vi "VIH HelpGen - Build Log Handler - Save Log File.vi"(6 "CHM status":T1, 7 "preparation error":errorcluster, 8 "error in":errorcluster, 9 "Menu Help status":T3, 10 "VI Help status":T4, 11 "Status":T2) -> (0 "error out":errorcluster)   [LabVIEW 2014]
doc: "::: VI Helpeks :::\nCopyright (c) 2000-2026 Konstantin Shifershteyn. All rights reserved."
uses:
  <vilib>/Utility/error.llb/DialogType.ctl
panel:
  # "VI Helpeks\nCopyright (c) 2012-2026 Konstantin Shifershteyn"
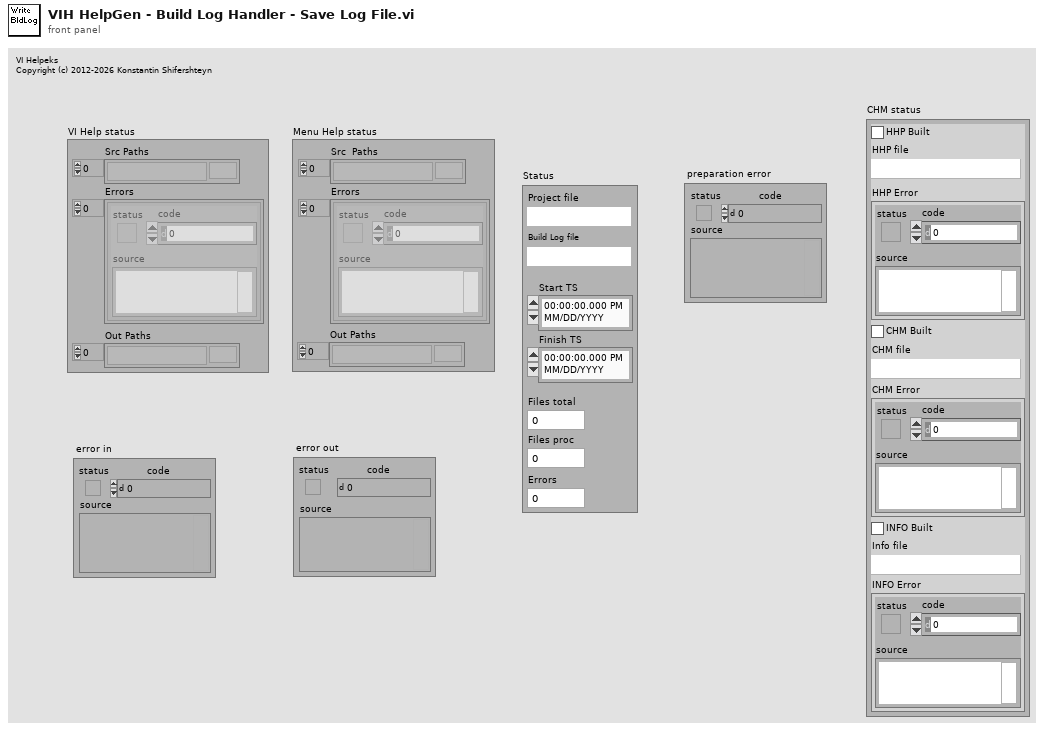
[diagram p1: front panel]
types:
  T1 = cluster{"HHP Built":bool, "HHP file":path, "HHP Error":errorcluster, "CHM Built":bool, "CHM file":path, "CHM Error":errorcluster, "INFO Built":bool, "Info file":path, "INFO Error":errorcluster}
  T2 = cluster{"Project file":path, "Build Log file":path, "Start TS":timestamp, "Finish TS":timestamp, "Files total":i32, "Files proc":i32, "Errors":i32}
  T3 = cluster{"Src  Paths":path[], "Errors":errorcluster[], "Out Paths":path[]}
  T4 = cluster{"Src Paths":path[], "Errors":errorcluster[], "Out Paths":path[]}
  T5 = enum16{"none", "LV description", "VH minimum", "VH extended"}
  T6 = typedef "DialogType.ctl" = u16
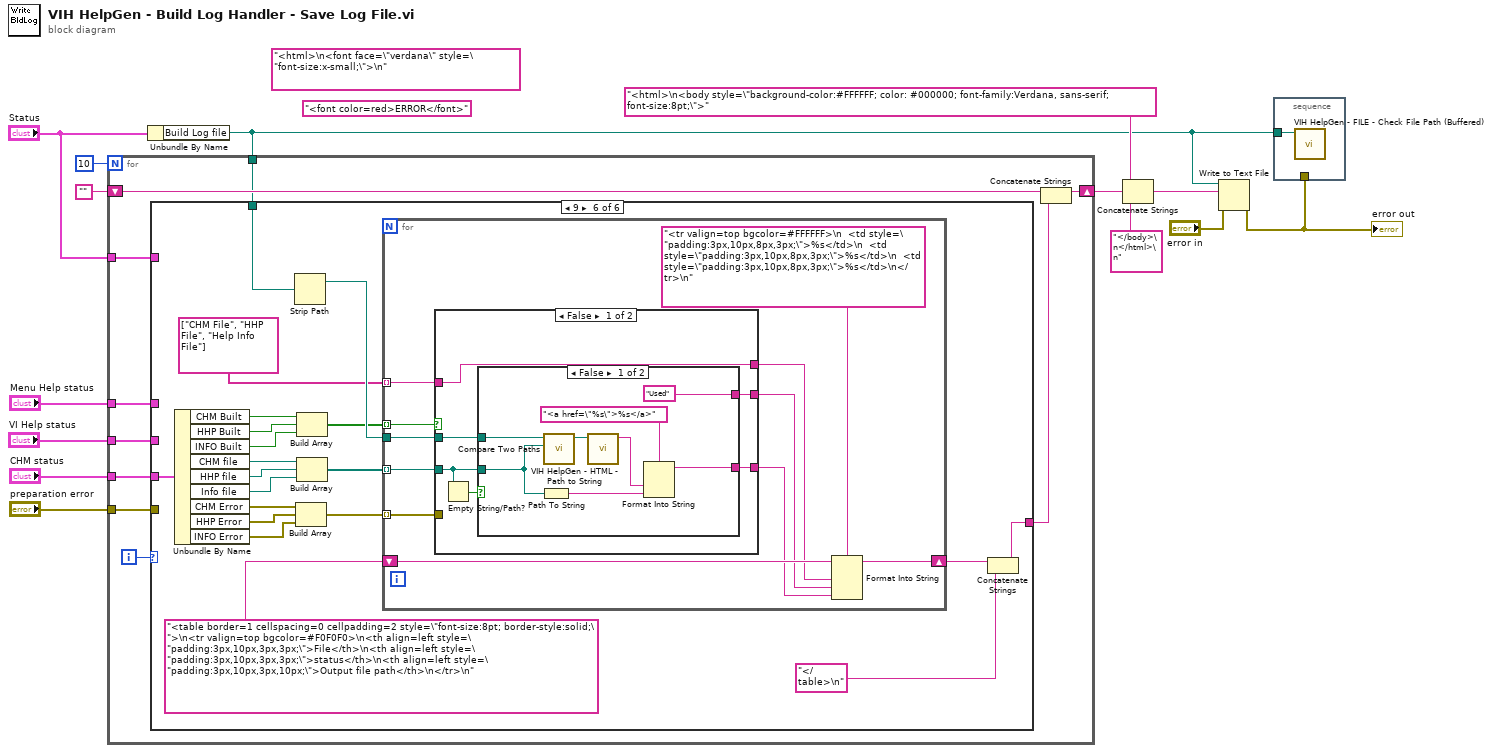
[diagram p0: block diagram]
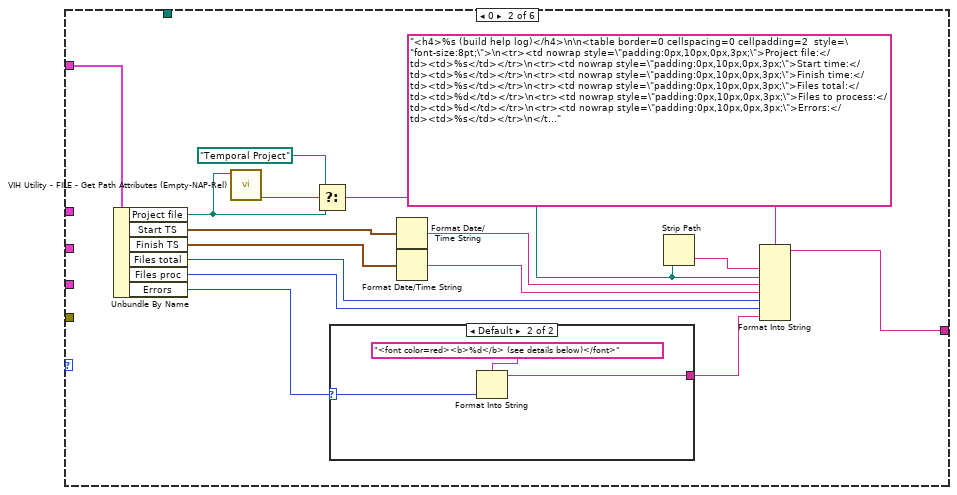
[diagram p3: hidden frame]
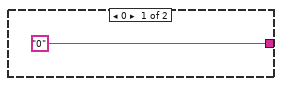
[diagram p4: hidden frame]
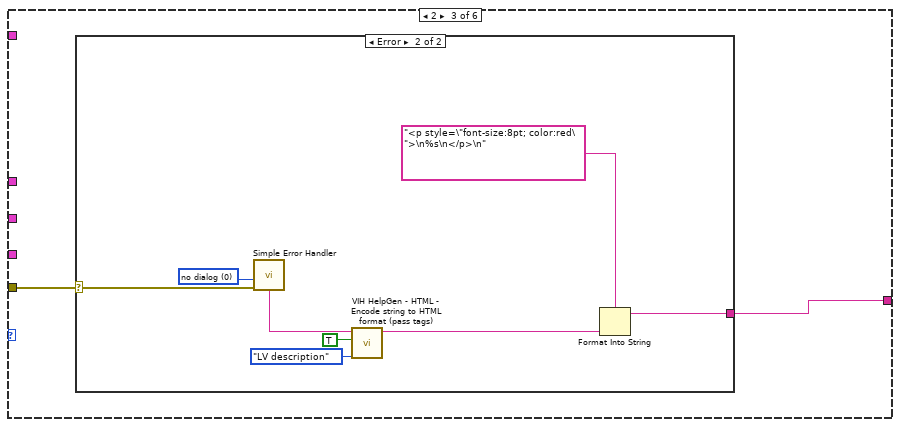
[diagram p5: hidden frame]
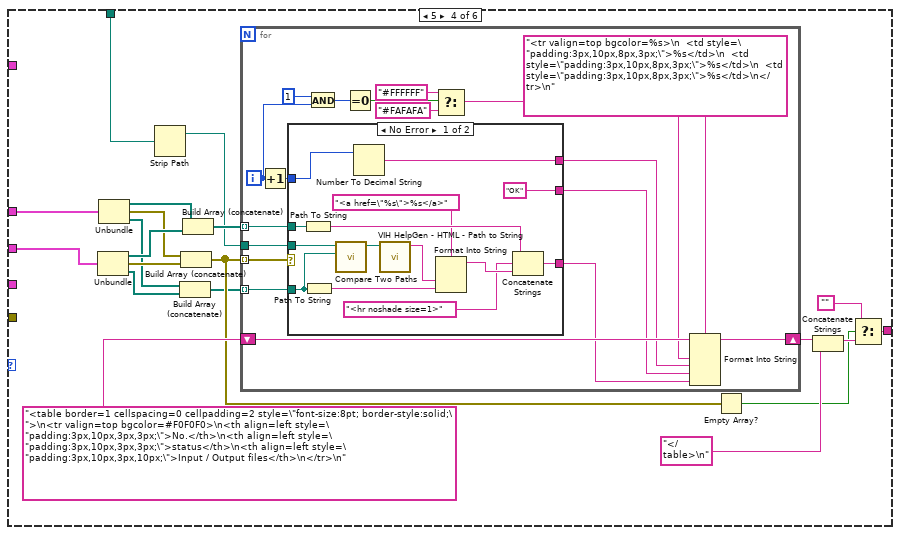
[diagram p7: hidden frame]
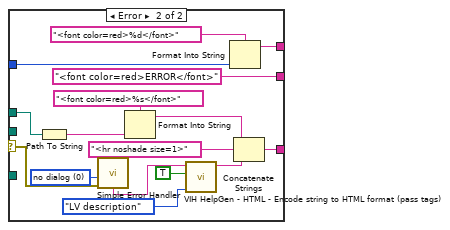
[diagram p8: hidden frame]
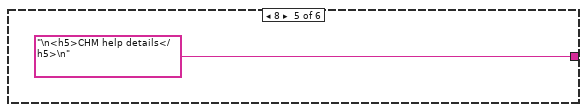
[diagram p9: hidden frame]
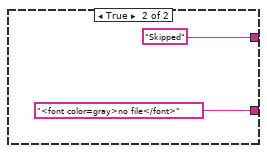
[diagram p10: hidden frame]
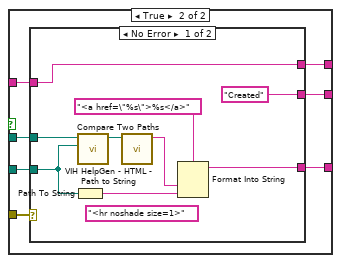
[diagram p11: hidden frame]
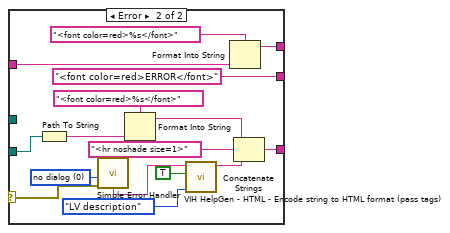
[diagram p12: hidden frame]
diagram:
  (unwired) "<font color=red>ERROR</font>"
  (unwired) "<html>\n<font face=\"verdana\" style=\"font-size:x-small;\">\n"
  n1 = Unbundle By Name("Status") -> ("Build Log file"=w4:path)
  n2 = for {
    N: 10 -> [_]
    shift-right: [w21] -> w14
    shift-left: "" -> [w23]
    tunnel: "Status" -> [w20]
    tunnel: "preparation error" -> [w19]
    tunnel: w4 -> [w18]
    tunnel: "CHM status" -> [w17]
    tunnel: "Menu Help status" -> [w16]
    tunnel: "VI Help status" -> [w15]
    i -> [w24]
    n3 = case shown="9" w24 {
      tunnel: [_ w39 w45 w65 "\n<h5>CHM help details</h5>\n" w131] -> w22
      tunnel: w20 -> [_ w32 _ _ _ _]
      tunnel: w19 -> [_ _ w46 _ _ _]
      tunnel: w18 -> [_ _ _ w58 _ w140]
      tunnel: w17 -> [_ _ _ _ _ w138]
      tunnel: w16 -> [_ _ _ w56 _ _]
      tunnel: w15 -> [_ _ _ w55 _ _]
      frame Default {
      }
      frame 0 {
        n4 = Unbundle By Name(w32) -> ("Project file"=w27:path, "Start TS"=w38:timestamp, "Finish TS"=w36:timestamp, "Files total"=w34:i32, "Files proc"=w33:i32, "Errors"=w30:i32)
        n5 = call "VIH Utility - FILE - Get Path Attributes (Empty-NAP-Rel).vi"("Path"=w27) -> ("Not A Path or Empty path"=w28:bool)  [unwired: 6 in, 4 out]
        n6 = Select(t=path "Temporal Project", s=w28, f=w27) -> (s? t:f=w25:path)
        n7 = case shown="Default" w30 {
          selector: w30 -> [_ w44]
          tunnel: ["0" w43] -> w29
          frame 0 {
          }
          frame Default {
            n8 = Format Into String(format string="<font color=red><b>%d</b> (see details below)</font>", w44) -> (resulting string=w43:string)  [unwired: 2 in, 1 out]
          }
        }
        n9 = Format Date/Time String(seconds (now)=w38) -> (date/time string=w37:string)  [unwired: 2 in]
        n10 = Format Date/Time String(seconds (now)=w36) -> (date/time string=w35:string)  [unwired: 2 in]
        n11 = Strip Path(path=w25) -> (name=w31:string)  [unwired: 1 out]
        n12 = Format Into String(format string="<h4>%s (build help log)</h4>\n\n<table border=0 cellspacing=0 cellpadding=2  style=\"font-size:8pt;\">\n<tr><td nowrap style=\"padding:0px,10px,0px,3px;\">Project file:</td><td>%s</td></tr>\n<tr><td nowrap style=\"padding:0px,10px,0px,3px;\">Start time:</td><td>%s</td></tr>\n<tr><td nowrap style=\"padding:0px,10px,0px,3px;\">Finish time:</td><td>%s</td></tr>\n<tr><td nowrap style=\"padding:0px,10px,0px,3px;\">Files total:</td><td>%d</td></tr>\n<tr><td nowrap style=\"padding:0px,10px,0px,3px;\">Files to process:</td><td>%d</td></tr>\n<tr><td nowrap style=\"padding:0px,10px,0px,3px;\">Errors:</td><td>%s</td></tr>\n</table>\n\n<h5>Build help details:</h5>\n", w31, w25, w37, w35, w34, w33, w29) -> (resulting string=w39:string)  [unwired: 2 in, 1 out]
      }
      frame 2 {
        n13 = case shown="Error" w46 {
          selector: w46 -> [_ w52]
          tunnel: [_ w49] -> w45
          frame No Error {
          }
          frame Error {
            w54 = T6 0 items=["no dialog", "OK message", "continue or stop message", "OK message + warnings", "continue/stop + warnings"] ("type of dialog (OK msg:1)")
            n14 = call <vilib>:"Simple Error Handler.vi"("type of dialog (OK msg:1)"=w54, "error in (no error)"=w52) -> ("message"=w53:string)  [unwired: 3 in, 4 out]
            n15 = call "VIH HelpGen - HTML - Encode string to HTML format (pass tags).vi"("HTML Tagset allowed"=T5."LV description" ("Tag set"), "Reject CR (F)"=TRUE, "string"=w53) -> ("HTML string"=w51:string)  [unwired: 8 in]
            n16 = Format Into String(format string="<p style=\"font-size:8pt; color:red\">\n%s\n</p>\n", w51) -> (resulting string=w49:string)  [unwired: 2 in, 1 out]
          }
        }
      }
      frame 5 {
        n17 = Unbundle(w55) -> ("Src Paths"=w70:path[], "Errors"=w68:errorcluster[], "Out Paths"=w60:path[])
        n18 = Unbundle(w56) -> ("Src  Paths"=w71:path[], "Errors"=w69:errorcluster[], "Out Paths"=w61:path[])
        n19 = Strip Path(path=w58) -> (stripped path=w57:path)  [unwired: 1 out]
        n20 = Build Array (concatenate)(w61, w60) -> (w59:path[])
        n21 = Build Array (concatenate)(w69, w68) -> (w63:errorcluster[])
        n22 = Build Array (concatenate)(w71, w70) -> (w67:path[])
        n23 = for {
          tunnel: w67 -> [w87] mode=indexing
          tunnel: w63 -> [w89] mode=indexing
          shift-right: [w90] -> w74
          shift-left: "<table border=1 cellspacing=0 cellpadding=2 style=\"font-size:8pt; border-style:solid;\">\n<tr valign=top bgcolor=#F0F0F0>\n<th align=left style=\"padding:3px,10px,3px,3px;\">No.</th>\n<th align=left style=\"padding:3px,10px,3px,3px;\">status</th>\n<th align=left style=\"padding:3px,10px,3px,10px;\">Input / Output files</th>\n</tr>\n" -> [w91]
          tunnel: w59 -> [w83] mode=indexing
          tunnel: w57 -> [w82]
          i -> [w81]
          n24 = Increment(x=w81) -> (x+1=w84:i32)
          n25 = case shown="No Error" w89 {
            selector: w89 -> [_ w118]
            tunnel: ["OK" ("f") "<font color=red>ERROR</font>"] -> w88
            tunnel: w87 -> [w105 w121]
            tunnel: [w99 w114] -> w86
            tunnel: [w103 w110] -> w85
            tunnel: w84 -> [w104 w109]
            tunnel: w83 -> [w96 _]
            tunnel: w82 -> [w95 _]
            frame No Error {
              n26 = Path To String(path=w105) -> (string=w98:string)
              n27 = Path To String(path=w96) -> (string=w102:string)
              n28 = call <vilib>:"Compare Two Paths.vi"("Path 2"=w96, "Path 1"=w95) -> ("Relative Path from 1 to 2"=w94:path)  [unwired: 6 in, 3 out]
              n29 = Number To Decimal String(number=w104) -> (decimal integer string=w103:string)  [unwired: 1 in]
              n30 = call "VIH HelpGen - HTML - Path to String.vi"("Path"=w94) -> ("String"=w93:string)  [unwired: 10 in]
              n31 = Format Into String(format string="<a href=\"%s\">%s</a>", w93, w102) -> (resulting string=w101:string)  [unwired: 2 in, 1 out]
              n32 = Concatenate Strings(w98, "<hr noshade size=1>" ("string"), w101) -> (w99:string)
            }
            frame Error {
              w117 = T6 0 items=["no dialog", "OK message", "continue or stop message", "OK message + warnings", "continue/stop + warnings"] ("type of dialog (OK msg:1)")
              n33 = Path To String(path=w121) -> (string=w120:string)
              n34 = call <vilib>:"Simple Error Handler.vi"("type of dialog (OK msg:1)"=w117, "error in (no error)"=w118) -> ("message"=w113:string)  [unwired: 3 in, 4 out]
              n35 = Format Into String(format string="<font color=red>%s</font>", w120) -> (resulting string=w116:string)  [unwired: 2 in, 1 out]
              n36 = call "VIH HelpGen - HTML - Encode string to HTML format (pass tags).vi"("HTML Tagset allowed"=T5."LV description" ("Tag set"), "Reject CR (F)"=TRUE, "string"=w113) -> ("HTML string"=w112:string)  [unwired: 8 in]
              n37 = Format Into String(format string="<font color=red>%d</font>", w109) -> (resulting string=w110:string)  [unwired: 2 in, 1 out]
              n38 = Concatenate Strings(w116, "<hr noshade size=1>" ("string"), w112) -> (w114:string)
            }
          }
          n39 = And(x=1, y=w81) -> (x .and. y?=w79:i32)
          n40 = Equal To 0?(x=w79) -> (x = 0?=w78:bool)
          n41 = Select(t="#FFFFFF", s=w78, f="#FAFAFA") -> (s? t:f=w75:string)
          n42 = Format Into String(format string="<tr valign=top bgcolor=%s>\n  <td style=\"padding:3px,10px,8px,3px;\">%s</td>\n  <td style=\"padding:3px,10px,8px,3px;\">%s</td>\n  <td style=\"padding:3px,10px,8px,3px;\">%s</td>\n</tr>\n", initial string=w91, w75, w85, w88, w86) -> (resulting string=w90:string)  [unwired: 1 in, 1 out]
        }
        n43 = Empty Array?(array=w63) -> (empty?=w62:bool)
        n44 = Concatenate Strings(w74, "</table>\n") -> (w66:string)
        n45 = Select(t="", s=w62, f=w66) -> (s? t:f=w65:string)
      }
      frame 8 {
      }
      frame 9 {
        n46 = Unbundle By Name(w138) -> ("CHM Built"=w129:bool, "HHP Built"=w137:bool, "INFO Built"=w124:bool, "CHM file"=w128:path, "HHP file"=w136:path, "Info file"=w135:path, "CHM Error"=w127:errorcluster, "HHP Error"=w134:errorcluster, "INFO Error"=w125:errorcluster)
        n47 = Strip Path(path=w140) -> (stripped path=w139:path)  [unwired: 1 out]
        n48 = Build Array(w127, w134, w125) -> (w133:errorcluster[])
        n49 = Build Array(w129, w137, w124) -> (w130:bool[])
        n50 = Build Array(w128, w136, w135) -> (w132:path[])
        n51 = for {
          tunnel: w132 -> [w149] mode=indexing
          tunnel: w133 -> [w151] mode=indexing
          shift-right: [w152] -> w143
          shift-left: "<table border=1 cellspacing=0 cellpadding=2 style=\"font-size:8pt; border-style:solid;\">\n<tr valign=top bgcolor=#F0F0F0>\n<th align=left style=\"padding:3px,10px,3px,3px;\">File</th>\n<th align=left style=\"padding:3px,10px,3px,3px;\">status</th>\n<th align=left style=\"padding:3px,10px,3px,10px;\">Output file path</th>\n</tr>\n" -> [w153]
          tunnel: w139 -> [w146]
          tunnel: w130 -> [w145] mode=indexing
          tunnel: string[] ["CHM File", "HHP File", "Help Info File"] -> [w144] mode=indexing
          n52 = case shown="False" w145 {
            tunnel: w151 -> [_ w177]
            tunnel: [w159 w176] -> w150
            tunnel: w149 -> [w155 w175]
            tunnel: [w158 w174] -> w148
            tunnel: [w160 w173] -> w147
            tunnel: w144 -> [w160 w172]
            tunnel: w146 -> [w156 w171]
            frame False {
              n53 = Empty String/Path?(string/path=w155) -> (empty?=w157:bool)
              n54 = case shown="False" w157 {
                tunnel: ["Used" "Skipped"] -> w159
                tunnel: [w161 "<font color=gray>no file</font>"] -> w158
                tunnel: w156 -> [w163 _]
                tunnel: w155 -> [w162 _]
                frame False {
                  n55 = Path To String(path=w162) -> (string=w167:string)
                  n56 = call <vilib>:"Compare Two Paths.vi"("Path 2"=w162, "Path 1"=w163) -> ("Relative Path from 1 to 2"=w165:path)  [unwired: 6 in, 3 out]
                  n57 = call "VIH HelpGen - HTML - Path to String.vi"("Path"=w165) -> ("String"=w164:string)  [unwired: 10 in]
                  n58 = Format Into String(format string="<a href=\"%s\">%s</a>", w164, w167) -> (resulting string=w161:string)  [unwired: 2 in, 1 out]
                }
                frame True {
                }
              }
            }
            frame True {
              n59 = case shown="No Error" w177 {
                selector: w177 -> [_ w198]
                tunnel: ["Created" ("f") "<font color=red>ERROR</font>"] -> w176
                tunnel: w175 -> [w180 w201]
                tunnel: [w178 w194] -> w174
                tunnel: [w179 w190] -> w173
                tunnel: w172 -> [w179 w189]
                tunnel: w171 -> [w183 _]
                frame No Error {
                  (unwired) "<hr noshade size=1>" ("string")
                  n60 = Path To String(path=w180) -> (string=w185:string)
                  n61 = call <vilib>:"Compare Two Paths.vi"("Path 2"=w180, "Path 1"=w183) -> ("Relative Path from 1 to 2"=w182:path)  [unwired: 6 in, 3 out]
                  n62 = call "VIH HelpGen - HTML - Path to String.vi"("Path"=w182) -> ("String"=w181:string)  [unwired: 10 in]
                  n63 = Format Into String(format string="<a href=\"%s\">%s</a>", w181, w185) -> (resulting string=w178:string)  [unwired: 2 in, 1 out]
                }
                frame Error {
                  w197 = T6 0 items=["no dialog", "OK message", "continue or stop message", "OK message + warnings", "continue/stop + warnings"] ("type of dialog (OK msg:1)")
                  n64 = Path To String(path=w201) -> (string=w200:string)
                  n65 = call <vilib>:"Simple Error Handler.vi"("type of dialog (OK msg:1)"=w197, "error in (no error)"=w198) -> ("message"=w193:string)  [unwired: 3 in, 4 out]
                  n66 = Format Into String(format string="<font color=red>%s</font>", w200) -> (resulting string=w196:string)  [unwired: 2 in, 1 out]
                  n67 = call "VIH HelpGen - HTML - Encode string to HTML format (pass tags).vi"("HTML Tagset allowed"=T5."LV description" ("Tag set"), "Reject CR (F)"=TRUE, "string"=w193) -> ("HTML string"=w192:string)  [unwired: 8 in]
                  n68 = Format Into String(format string="<font color=red>%s</font>", w189) -> (resulting string=w190:string)  [unwired: 2 in, 1 out]
                  n69 = Concatenate Strings(w196, "<hr noshade size=1>" ("string"), w192) -> (w194:string)
                }
              }
            }
          }
          n70 = Format Into String(format string="<tr valign=top bgcolor=#FFFFFF>\n  <td style=\"padding:3px,10px,8px,3px;\">%s</td>\n  <td style=\"padding:3px,10px,8px,3px;\">%s</td>\n  <td style=\"padding:3px,10px,8px,3px;\">%s</td>\n</tr>\n", initial string=w153, w147, w150, w148) -> (resulting string=w152:string)  [unwired: 1 in, 1 out]
        }
        n71 = Concatenate Strings(w143, "</table>\n") -> (w131:string)
      }
    }
    n72 = Concatenate Strings(w23, w22) -> (w21:string)
  }
  n73 = Concatenate Strings("<html>\n<body style=\"background-color:#FFFFFF; color: #000000; font-family:Verdana, sans-serif; font-size:8pt;\">", w14, "</body>\n</html>\n") -> (w10:string)
  n74 = Write to Text File(file (use dialog)=w4, text=w10, error in="error in") -> (error out=w5:errorcluster)  [unwired: 1 in, 2 out]
  "error out" <- w5
  n75 = stacked-sequence {
    tunnel: w4 -> [w203]
    tunnel: w5 -> [_]
    frame #0 {
      n76 = call "VIH HelpGen - FILE - Check File Path (Buffered).vi"("File Path"=w203) -> ()  [unwired: 9 in, 2 out]
    }
  }
